vi "AssertAlmostEqual_Tests.vi"(11 "error in":errorcluster) -> (15 "error out":errorcluster)   [LabVIEW 2016, in "DronaTest.lvlib"]
uses:
  DronaTest.lvlib
  APIs/Assert/AssertControlValue/AlmostEqual.vi
  <vilib>/addons/_JKI Toolkits/Caraya/classes/Assert/Assert Almost Equal_Float.vi
  <vilib>/addons/_JKI Toolkits/Caraya/classes/Assert/Assert Error.vi
  <vilib>/addons/_JKI Toolkits/Caraya/classes/Test/Test.lvclass
  Drona.lvlib
  APIs/Assert/AssertControlValue/AssertControlValue.lvlib
  <vilib>/addons/_JKI Toolkits/Caraya/classes/Assert/Assert.lvclass
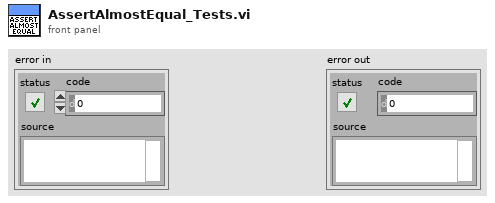
[diagram p1: front panel]
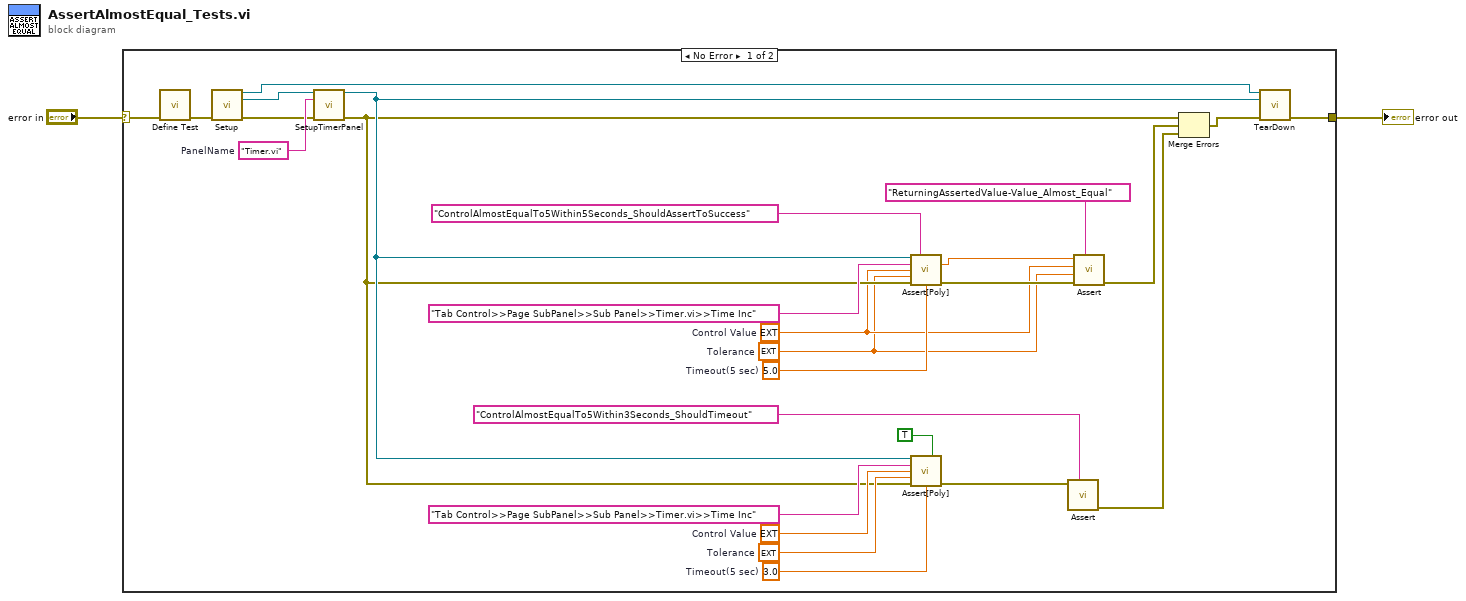
[diagram p0: block diagram]
diagram:
  n1 = case shown="No Error" "error in" {
    selector: "error in" -> [w29 w30]
    tunnel: [w19 w30] -> w1
    frame No Error {
      w17 = "Timer.vi"  # PanelName
      w22 = ext 0.5  # Tolerance
      w4 = ext 0.5  # Tolerance
      w26 = 3.0  # Timeout(5 sec)
      w25 = ext 5.0  # Control Value
      w27 = 5.0  # Timeout(5 sec)
      w5 = ext 5.0  # Control Value
      n2 = call <vilib>:"Define Test.vi"("error in (no error)"=w29) -> ("error out"=w21:errorcluster)  [unwired: 9 in, 1 out]
      n3 = call "Setup.vi"("error in"=w21) -> ("Application Ref"=w18:refnum<vi>, "VI out"=w15:refnum<vi>, "error out"=w16:errorcluster)  [unwired: 12 in]
      n4 = call "SetupTimerPanel.vi"("VI in"=w15, "Item Name"=w17, "error in (no error)"=w16) -> ("VI out"=w14:refnum<vi>, "error out"=w13:errorcluster)  [unwired: 11 in]
      n5 = call-poly "Assert[Poly].vi"("VI Reference In"=w14, "Test Label"="ControlAlmostEqualTo5Within5Seconds_ShouldAssertToSuccess" ("string"), "Control Path"="Tab Control>>Page SubPanel>>Sub Panel>>Timer.vi>>Time Inc", "Control Value"=w5, "Tolerance"=w4, "Error In"=w13, "Timeout(5 sec)"=w27) -> ("Asserted Value"=w6:ext, "Error Out"=w8:errorcluster)  [unwired: 6 in, 1 out]
      n6 = call-poly "Assert[Poly].vi"("VI Reference In"=w14, "Assert Only? (F)"=TRUE, "Control Path"="Tab Control>>Page SubPanel>>Sub Panel>>Timer.vi>>Time Inc", "Control Value"=w25, "Tolerance"=w22, "Error In"=w13, "Timeout(5 sec)"=w26) -> ("Error Out"=w9:errorcluster)  [unwired: 6 in, 2 out]
      n7 = call-poly <vilib>:"Assert.vi"("Label"="ControlAlmostEqualTo5Within3Seconds_ShouldTimeout" ("string"), "Error?"=w9) -> ("error out"=w11:errorcluster)  [unwired: 8 in, 1 out]
      n8 = call-poly <vilib>:"Assert.vi"("Label"="ReturningAssertedValue-Value_Almost_Equal", "error in (no error)"=w8, "Tolerance"=w4, "Y"=w5, "X"=w6) -> ("error out"=w7:errorcluster)  [unwired: 5 in, 1 out]
      n9 = Merge Errors(w13, w7, w11) -> (w20:errorcluster)
      n10 = call "TearDown.vi"("Application Ref"=w18, "VI in"=w14, "error in (no error)"=w20) -> ("error out"=w19:errorcluster)  [unwired: 12 in]
    }
    frame Error {
    }
  }
  "error out" <- w1
